vi "BasicControlPathAndType_Tests.vi"(11 "error in":errorcluster) -> (15 "error out":errorcluster)   [LabVIEW 2016, in "DronaTest.lvlib"]
uses:
  DronaTest.lvlib
  APIs/Stimulus/ControlValue/ValueSignalByPathString.vi
  APIs/Assert/AssertControlValue/Equal.vi
  <vilib>/addons/_JKI Toolkits/Caraya/classes/Test/Test.lvclass
  Drona.lvlib
  APIs/Assert/AssertControlValue/AssertControlValue.lvlib
  APIs/Stimulus/ControlValue/ControlValue.lvlib
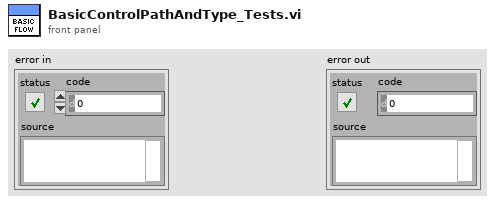
[diagram p1: front panel]
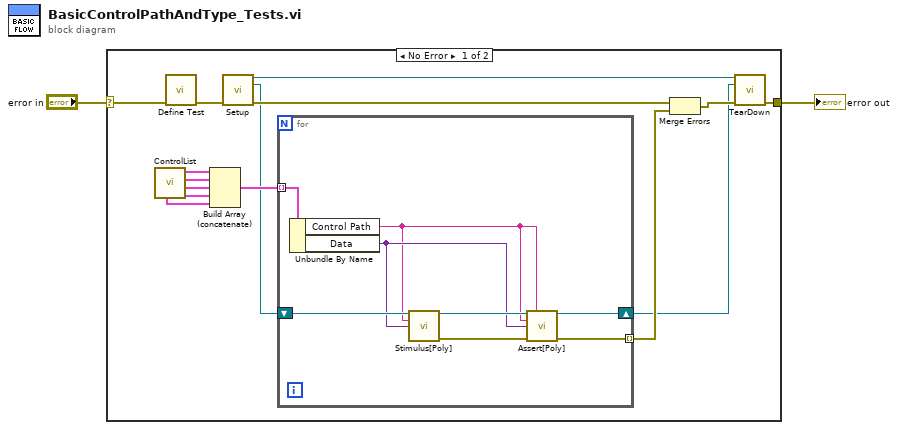
[diagram p0: block diagram]
diagram:
  n1 = case shown="No Error" "error in" {
    selector: "error in" -> [w16 w26]
    tunnel: [w6 w26] -> w1
    frame No Error {
      n2 = call "ControlList.vi"() -> ("Tab Control"=w9:cluster{"Control Path":string, "Data":variant}[], "BigCluster"=w10:cluster{"Control Path":string, "Data":variant}[], "Cluster"=w11:cluster{"Control Path":string, "Data":variant}[], "Basic"=w14:cluster{"Control Path":string, "Data":variant}[], "BasicArray"=w8:cluster{"Control Path":string, "Data":variant}[])  [unwired: 6 in, 1 out]
      n3 = call <vilib>:"Define Test.vi"("error in (no error)"=w16) -> ("error out"=w13:errorcluster)  [unwired: 9 in, 1 out]
      n4 = Build Array (concatenate)(w14, w11, w10, w9, w8) -> (w12:cluster{"Control Path":string, "Data":variant}[])
      n5 = call "Setup.vi"("error in (no error)"=w13) -> ("Application Ref"=w3:refnum<vi>, "VI out"=w4:refnum<vi>, "error out"=w7:errorcluster)  [unwired: 12 in]
      n6 = for {
        shift-right: [w25] -> w5
        shift-left: w4 -> [w21]
        tunnel: [w18] -> w17 mode=indexing
        tunnel: w12 -> [w22] mode=indexing
        n7 = Unbundle By Name(w22) -> ("Control Path"=w19:string, "Data"=w20:variant)
        n8 = call-poly "Stimulus[Poly].vi"("VI Reference In"=w21, "Control Path"=w19, "Value (Signaling)"=w20) -> ("VI Reference Out"=w23:refnum<vi>, "error out"=w24:errorcluster)  [unwired: 11 in]
        n9 = call-poly "Assert[Poly].vi"("VI Reference In"=w23, "Test Label"=w19, "Control Path"=w19, "Control Value"=w20, "Error In"=w24) -> ("VI Reference Out"=w25:refnum<vi>, "Error Out"=w18:errorcluster)  [unwired: 8 in, 1 out]
      }
      n10 = Merge Errors(w7, w17) -> (w15:errorcluster)
      n11 = call "TearDown.vi"("Application Ref"=w3, "VI in"=w5, "error in (no error)"=w15) -> ("error out"=w6:errorcluster)  [unwired: 12 in]
    }
    frame Error {
    }
  }
  "error out" <- w1
